vi "initialize Mast Device.vi"(8 "error in (no error)":errorcluster, 10 "VISA resource name":refnum<visa-resource-name>, 11 "CO3000 in":refnum<class "CO3000.lvclass">) -> (0 "error out":errorcluster, 3 "CO3000 out":refnum<class "CO3000.lvclass">)   [LabVIEW 2023, in "Turn Table and Mast.lvlib" / "CO3000.lvclass"]
uses:
  CO3000.lvclass
  CO3000.lvclass/CO3000.ctl
  <vilib>/ErrorRing/Error Ring.xnode
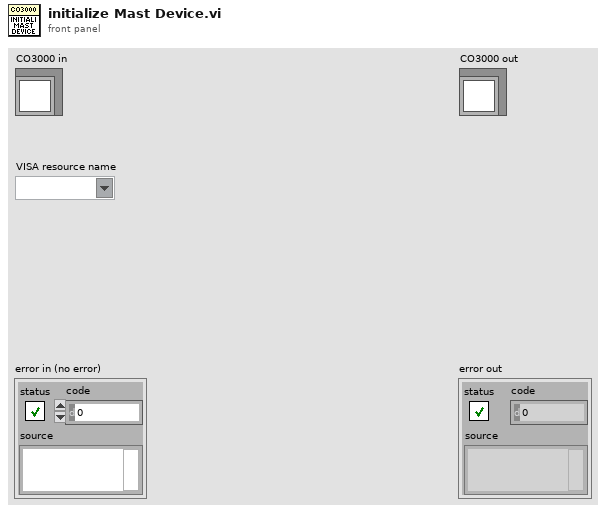
[diagram p1: front panel]
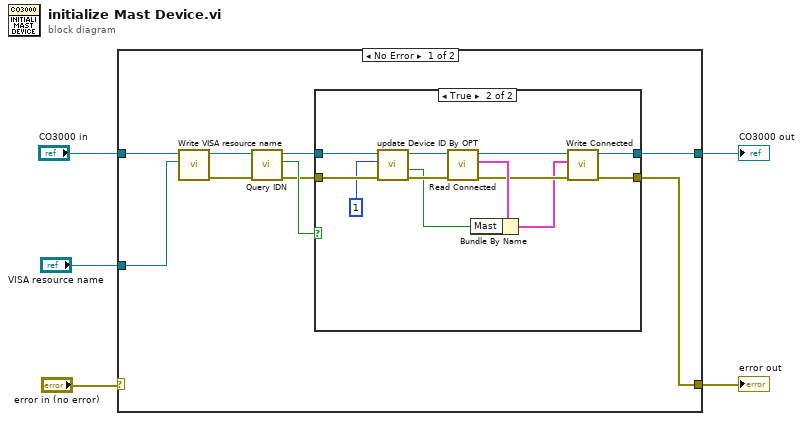
[diagram p0: block diagram]
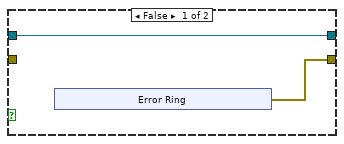
[diagram p2: hidden frame]
diagram:
  n1 = case shown="No Error" "error in (no error)" {
    selector: "error in (no error)" -> [_ w30]
    tunnel: "CO3000 in" -> [w14 w31]
    tunnel: [w7 w31] -> w4
    tunnel: [w6 w30] -> w2
    tunnel: "VISA resource name" -> [w13 _]
    frame No Error {
      n2 = call "Write VISA resource name.vi"("VISA resource name"=w13, "CO3000 in"=w14) -> ("error out"=w11:errorcluster, "CO3000 out"=w12:refnum<class "CO3000.lvclass">)  [unwired: 8 in]
      n3 = call-dynamic "Query IDN.vi"("error in (no error)"=w11, "CO3000 in"=w12) -> ("error out"=w8:errorcluster, "Connected?"=w9:bool, "CO3000 out"=w10:refnum<class "CO3000.lvclass">)  [unwired: 7 in]
      n4 = case shown="True" w9 {
        tunnel: w10 -> [w16 w29]
        tunnel: w8 -> [_ w28]
        tunnel: [w16 w20] -> w7
        tunnel: [w15 w19] -> w6
        frame False {
          n5 = xnode "Error Ring"() -> ("error out"=w15:errorcluster)
        }
        frame True {
          n6 = call "update Device ID By OPT.vi"("error in (no error)"=w28, "Mast Index"=1, "CO3000 in"=w29) -> ("error out"=w24:errorcluster, "Mast Available?"=w18:bool, "CO3000 out"=w25:refnum<class "CO3000.lvclass">)  [unwired: 5 in, 1 out]
          n7 = call "Read Connected.vi"("error in (no error)"=w24, "CO3000 in"=w25) -> ("error out"=w22:errorcluster, "Connected"=w26:cluster{"Mast":bool, "Turn Table":bool}, "CO3000 out"=w23:refnum<class "CO3000.lvclass">)  [unwired: 7 in]
          n8 = Bundle By Name(cluster=w26, "Mast"=w18) -> (w21:cluster{"Mast":bool, "Turn Table":bool})
          n9 = call "Write Connected.vi"("error in (no error)"=w22, "Connected"=w21, "CO3000 in"=w23) -> ("error out"=w19:errorcluster, "CO3000 out"=w20:refnum<class "CO3000.lvclass">)  [unwired: 7 in]
        }
      }
    }
    frame Error {
    }
  }
  "error out" <- w2
  "CO3000 out" <- w4
